vi "Init.vi"(8 "error in (no error)":errorcluster, 11 "Data in":refnum<class "CTI_TCP_Bus.lvclass">) -> (0 "error out":errorcluster, 3 "Data out":refnum<class "CTI_TCP_Bus.lvclass">)   [LabVIEW 2021, in "CTI_TCP_Bus.lvclass"]
doc: "Abstract Data Classes 2.1.1.12\nTim Streeter - TSA\nCopyright (c) 2024, TSAOmni-Bus 2.0.1.6\nTim - TSA\nCopyright (c) 2024, TSA"
uses:
  CTI_TCP_Bus.lvclass
  C:/TSA/CTI_Bus/Source/Parent/CTI_Bus.lvclass
  Parent/CTI_Bus.lvclass/CTI_Bus.ctl
  Parent/Properties/Read Error Checking.vi
  Parent/Properties/Read VISA resource name.vi
  Parent/Properties/Write Session.vi
  Parent/Properties/Write Identity.vi
  Parent/CTI_Bus.lvclass
  <vilib>/CTI/CTI Drivers/CTI/VisaComms/VisaComms.lvclass
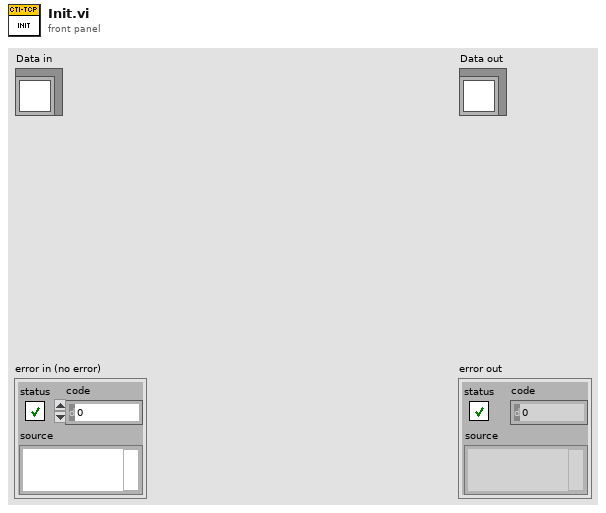
[diagram p1: front panel]
types:
  T1 = typedef "CTI.lvlib/Error Reporting.ctl" = enum16{"Minimal", "Moderate", "Full"}
  T2 = typedef "CTI.lvlib/Identity.ctl" = cluster{"Vendor":string, "Model":string, "Serial":string, "Version":string}
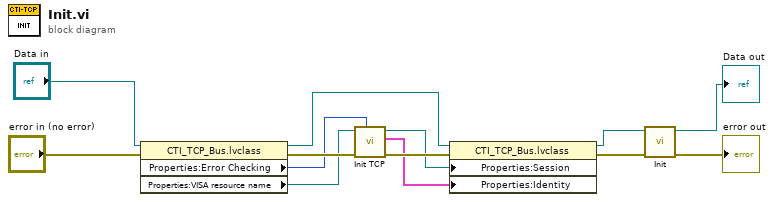
[diagram p0: block diagram]
diagram:
  n1 = property class="CTI_TCP_Bus.lvclass"(reference="Data in", error in="error in (no error)") -> (reference out=w10:refnum<class "CTI_TCP_Bus.lvclass">, error out=w13:errorcluster, "Properties:Error Checking"=w9:T1, "Properties:VISA resource name"=w12:refnum<visa-resource-name>)
  n2 = call <vilib>:"Init TCP.vi"("Error Checking (Full)"=w9, "error in (no error)"=w13, "VISA resource name"=w12) -> ("error out"=w11:errorcluster, "Identity"=w7:T2, "Session"=w8:refnum<class "Session.lvclass">)  [unwired: 6 in]
  n3 = property class="CTI_TCP_Bus.lvclass"(reference=w10, error in=w11, "Properties:Session"=w8, "Properties:Identity"=w7) -> (reference out=w2:refnum<class "CTI_TCP_Bus.lvclass">, error out=w4:errorcluster)
  n4 = call-parent "Init.vi"("error in (no error)"=w4, "Data in"=w2) -> ("error out"=→"error out":errorcluster, "Data out"=→"Data out":refnum<class "CTI_TCP_Bus.lvclass">)  [unwired: 8 in]
